vi "SPARK Get Limit Switch Config.vi"   [LabVIEW 2027]
doc: "Get the configuration of a limit switch connected to the data port of the SPARK."
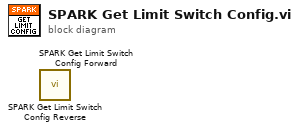
[diagram p0: block diagram]
diagram:
  n1 = call <vilib>:"SPARK Get Limit Switch Config Reverse.vi"() -> ()  [unwired: 6 in, 6 out]
  n2 = call <vilib>:"SPARK Get Limit Switch Config Forward.vi"() -> ()  [unwired: 6 in, 6 out]
